vi "Frame.Settings.vi"(6 "Action":enum8{"Get", "Set"}(ring), 8 "error in (no error)":errorcluster, 10 "Frame.Settings":T1={"ID"=0, "Disable Transmission"=FALSE, "Disable Transmission Ref"=18446744073709551615, "Transmit Trigger"=enum."Channel value change", "Transmit Trigger Ref"=18446744073709551615} {"Transmit Trigger Ref" format="%.0x"; "Disable Transmission Ref" format="%.0x"}, 11 "Item Ref in":T2 format="%.0x") -> (0 "error out":errorcluster, 2 "Frame.Settings":T1={"ID"=0, "Disable Transmission"=FALSE, "Disable Transmission Ref"=18446744073709551615, "Transmit Trigger"=enum."Channel value change", "Transmit Trigger Ref"=18446744073709551615} {"Transmit Trigger Ref" format="%.0x"; "Disable Transmission Ref" format="%.0x"}, 3 "Item Ref out":T2 format="%.0x")   [LabVIEW 2025, in "Protection and Counter Addon System Explorer.lvlib"]
uses:
  Protection and Counter Addon System Explorer.lvlib
  <vilib>/NI VeriStand/Custom Device API/Custom Device Item Ref.ctl
  Types/Frame Settings.ctl
  Types/Event Trigger Type.ctl
  Addon Shared/SubVIs/GUID Lookup.vi
  Addon Shared/Protection and Counter Addon Shared.lvlib
  <vilib>/NI/NI VeriStand Advanced SysDef API/SysDef API/Advanced System Definition.lvlib
  <vilib>/NI/NI VeriStand Advanced SysDef API/_SubVIs/SysDef.Property.Get.U32.vi
  <vilib>/NI/NI VeriStand Advanced SysDef API/_SubVIs/SysDef.Property.Get.Boolean.vi
  <vilib>/NI/NI VeriStand Advanced SysDef API/_SubVIs/SysDef.Property.Set.U32.vi
  <vilib>/NI/NI VeriStand Advanced SysDef API/_SubVIs/SysDef.Property.Set.Boolean.vi
  <vilib>/NI/NI VeriStand Advanced SysDef API/_SubVIs/SysDef.Property.Set.Node.vi
  <vilib>/NI/NI VeriStand Advanced SysDef API/_SubVIs/SysDef.Search.Parent.vi
  <vilib>/NI/NI VeriStand Advanced SysDef API/_SubVIs/SysDef.Property.Get.Node.vi
  <vilib>/NI VeriStand/Custom Device API/Custom Device API.lvlib
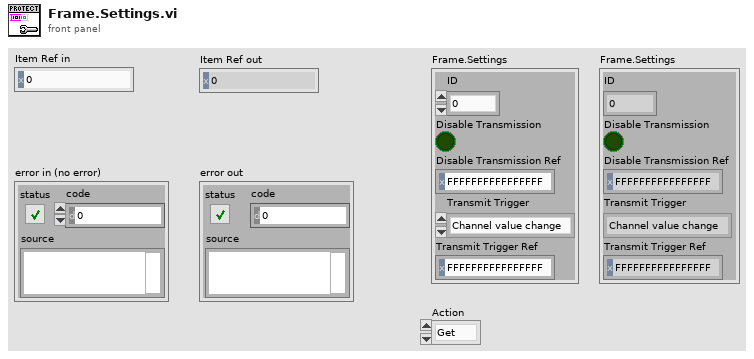
[diagram p1: front panel]
types:
  T1 = typedef "Protection and Counter Addon System Explorer.lvlib/Frame Settings.ctl" = cluster{"ID":u32, "Disable Transmission":bool, "Disable Transmission Ref":T2, "Transmit Trigger":T3, "Transmit Trigger Ref":T2}
  T2 = typedef "Custom Device API.lvlib/Custom Device Item Ref.ctl" = u64
  T3 = typedef "Protection and Counter Addon System Explorer.lvlib/Event Trigger Type.ctl" = enum16{"Channel value change", "Trigger channel (not zero)", "Channel value change or trigger channel (not zero)", "Trigger channel (any value change)", "Channel value change or trigger channel (any value change)"}
  T4 = typedef "Advanced System Definition.lvlib/TreeItem.Info.ctl" = cluster{"Name":string, "Description":string, "GUID":string, "Is Channel":bool, "Channel":T5, "Is Waveform":bool, "Waveform":T7}
  T5 = typedef "Custom Device API.lvlib/Custom Device Channel.ctl" = cluster{"Type":T6, "Units":string, "Default Value":dbl, "Faultable":bool, "Scalable":bool}
  T6 = typedef "Custom Device API.lvlib/Custom Device Channel Type.ctl" = enum16{"Input", "Output"}
  T7 = typedef "Custom Device API.lvlib/Custom Device Waveform.ctl" = cluster{"Data Type":T8, "Units":string}
  T8 = typedef "Custom Device API.lvlib/Custom Device Waveform DataType.ctl" = enum16{"Double", "Complex Double"}
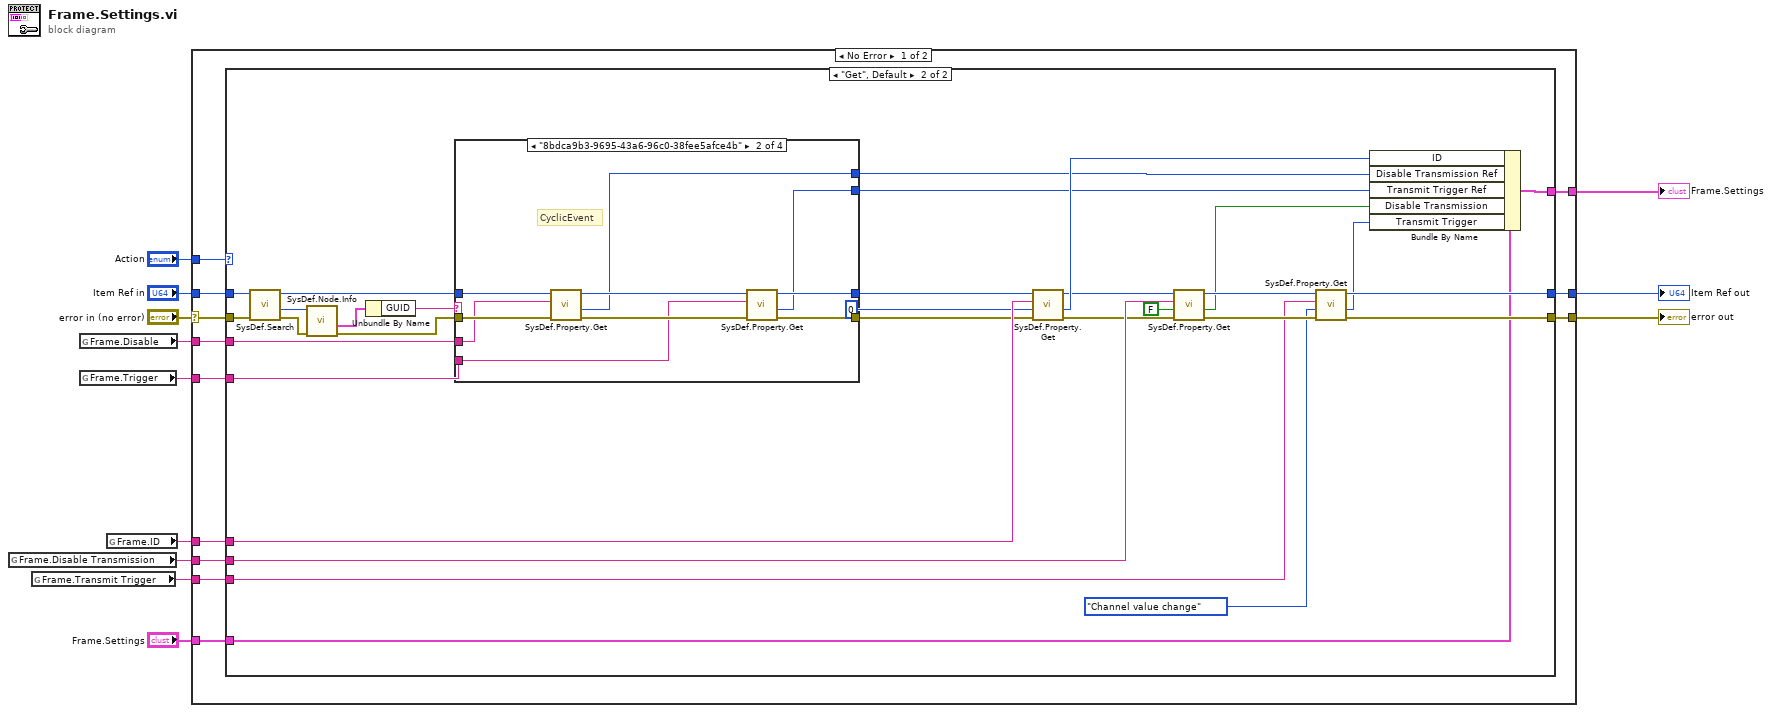
[diagram p0: block diagram]
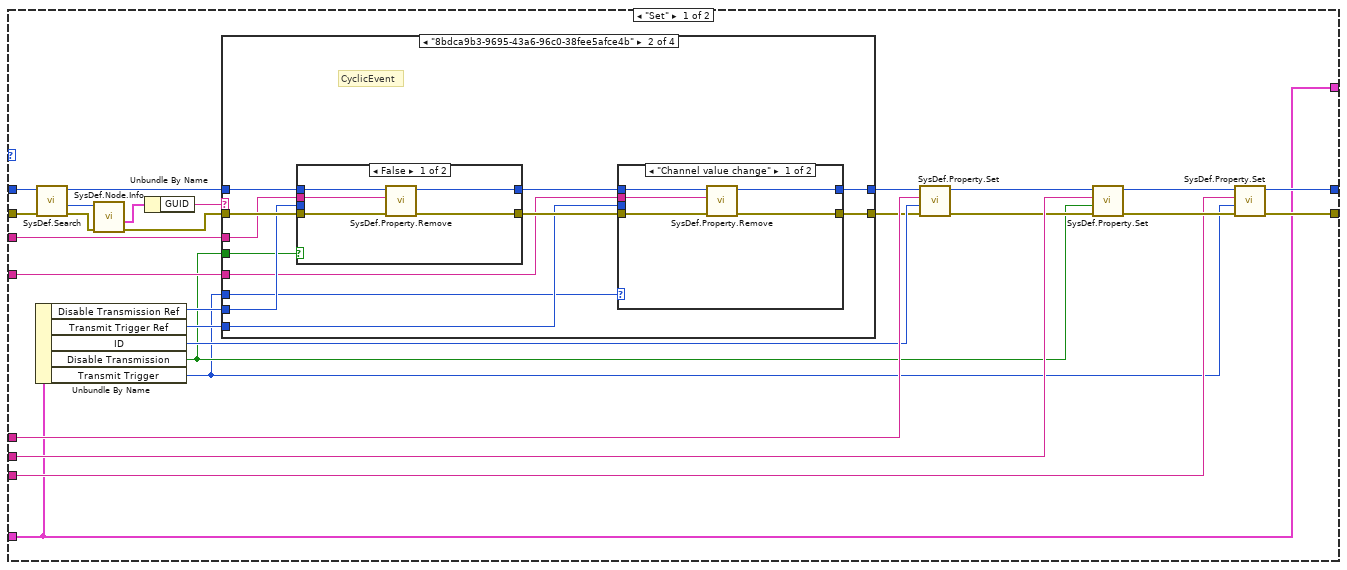
[diagram p2: hidden frame]
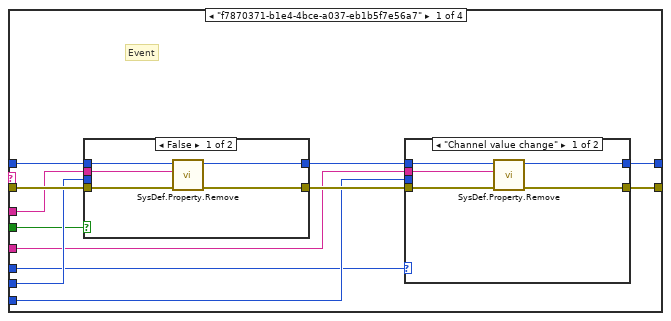
[diagram p3: hidden frame]
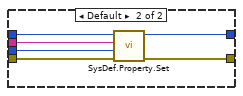
[diagram p4: hidden frame]
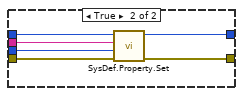
[diagram p5: hidden frame]
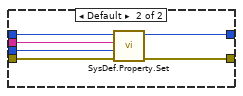
[diagram p6: hidden frame]
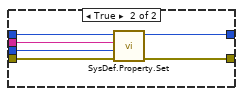
[diagram p7: hidden frame]
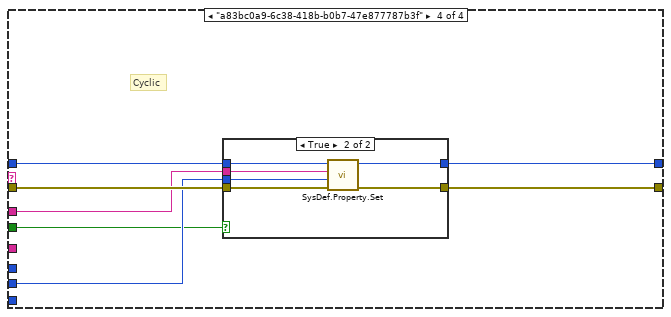
[diagram p9: hidden frame]
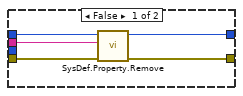
[diagram p10: hidden frame]
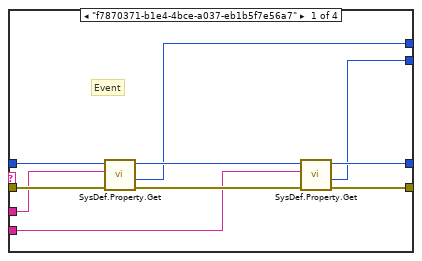
[diagram p11: hidden frame]
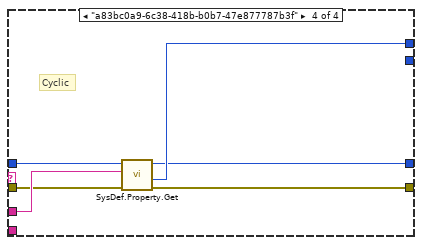
[diagram p13: hidden frame]
diagram:
  n1 = global read "GUID Lookup.vi" "Frame.Disable Transmission"() -> (w4:string)
  n2 = global read "GUID Lookup.vi" "Frame.Transmit Trigger"() -> (w5:string)
  n3 = global read "GUID Lookup.vi" "Frame.Disable"() -> (w1:string)
  n4 = global read "GUID Lookup.vi" "Frame.Trigger"() -> (w2:string)
  n5 = global read "GUID Lookup.vi" "Frame.ID"() -> (w3:string)
  n6 = case shown="No Error" "error in (no error)" {
    selector: "error in (no error)" -> [w15 w199]
    tunnel: "Item Ref in" -> [w24 w198]
    tunnel: w3 -> [w23 _]
    tunnel: w1 -> [w22 _]
    tunnel: w2 -> [w21 _]
    tunnel: [w20 w199] -> w11
    tunnel: [w19 w198] -> w10
    tunnel: [w18 _] -> w9
    tunnel: w5 -> [w17 _]
    tunnel: w4 -> [w16 _]
    tunnel: "Frame.Settings" -> [w14 _]
    tunnel: "Action" -> [w13 _]
    frame No Error {
      n7 = case shown="\"Get\", Default" w13 {
        tunnel: w24 -> [w37 w149]
        tunnel: w23 -> [w50 w169]
        tunnel: w22 -> [w34 w144]
        tunnel: w21 -> [w33 w143]
        tunnel: [w47 w165] -> w20
        tunnel: [w46 w164] -> w19
        tunnel: [w43 w157] -> w18
        tunnel: w17 -> [w45 w163]
        tunnel: w16 -> [w44 w162]
        tunnel: w15 -> [w36 w146]
        tunnel: w14 -> [w43 w158]
        frame "Set" {
          n8 = Unbundle By Name(w43) -> ("Disable Transmission Ref"=w28:T2, "Transmit Trigger Ref"=w27:T2, "ID"=w42:u32, "Disable Transmission"=w26:bool, "Transmit Trigger"=w25:T3)
          n9 = call-poly <vilib>:"SysDef.Search.vi"("error in (no error)"=w36, "nodeID"=w37) -> ("error out"=w32:errorcluster, "Value out"=w39:u64, "nodeID out"=w38:u64)  [unwired: 6 in, 1 out]
          n10 = call <vilib>:"SysDef.Node.Info.vi"("error in (no error)"=w32, "nodeID"=w39) -> ("error out"=w35:errorcluster, "Item Info"=w40:T4)  [unwired: 6 in, 2 out]
          n11 = Unbundle By Name(w40) -> ("GUID"=w41:string)
          n12 = case shown="\"8bdca9b3-9695-43a6-96c0-38fee5afce4b\"" w41 {
            tunnel: w35 -> [w62 w96 w120 w127]
            tunnel: [w52 w86 w120 w122] -> w31
            tunnel: w34 -> [w61 w95 _ w125]
            tunnel: w33 -> [w55 w89 _ _]
            tunnel: w38 -> [w60 w94 w119 w124]
            tunnel: [w53 w87 w119 w123] -> _
            tunnel: w28 -> [w59 w93 _ w126]
            tunnel: w27 -> [w56 w90 _ _]
            tunnel: w26 -> [w58 w92 _ w121]
            tunnel: w25 -> [w51 w85 _ _]
            frame "f7870371-b1e4-4bce-a037-eb1b5f7e56a7" {
              # "Event"
              n13 = case shown="False" w58 {
                tunnel: [w74 w84] -> w54
                tunnel: [w75 w83] -> w57
                tunnel: w62 -> [w76 w82]
                tunnel: w61 -> [w77 w81]
                tunnel: w60 -> [w78 w80]
                tunnel: w59 -> [_ w79]
                frame False {
                  n14 = call <vilib>:"SysDef.Property.Remove.vi"("error in (no error)"=w76, "Property Name"=w77, "nodeID"=w78) -> ("error out"=w75:errorcluster, "nodeID out"=w74:u64)  [unwired: 6 in, 1 out]
                }
                frame True {
                  n15 = call-poly <vilib>:"SysDef.Property.Set.vi"("error in (no error)"=w82, "Value"=w79, "Property Name"=w81, "nodeID"=w80) -> ("error out"=w83:errorcluster, "nodeID out"=w84:u64)  [unwired: 6 in]
                }
              }
              n16 = case shown="\"Channel value change\"" w51 {
                tunnel: [w63 w73] -> w53
                tunnel: [w64 w72] -> w52
                tunnel: w57 -> [w65 w71]
                tunnel: w55 -> [w66 w70]
                tunnel: w54 -> [w67 w69]
                tunnel: w56 -> [_ w68]
                frame "Channel value change" {
                  n17 = call <vilib>:"SysDef.Property.Remove.vi"("error in (no error)"=w65, "Property Name"=w66, "nodeID"=w67) -> ("error out"=w64:errorcluster, "nodeID out"=w63:u64)  [unwired: 6 in, 1 out]
                }
                frame Default {
                  n18 = call-poly <vilib>:"SysDef.Property.Set.vi"("error in (no error)"=w71, "Value"=w68, "Property Name"=w70, "nodeID"=w69) -> ("error out"=w72:errorcluster, "nodeID out"=w73:u64)  [unwired: 6 in]
                }
              }
            }
            frame "8bdca9b3-9695-43a6-96c0-38fee5afce4b" {
              # "CyclicEvent"
              n19 = case shown="False" w92 {
                tunnel: [w108 w118] -> w88
                tunnel: [w109 w117] -> w91
                tunnel: w96 -> [w110 w116]
                tunnel: w95 -> [w111 w115]
                tunnel: w94 -> [w112 w114]
                tunnel: w93 -> [_ w113]
                frame False {
                  n20 = call <vilib>:"SysDef.Property.Remove.vi"("error in (no error)"=w110, "Property Name"=w111, "nodeID"=w112) -> ("error out"=w109:errorcluster, "nodeID out"=w108:u64)  [unwired: 6 in, 1 out]
                }
                frame True {
                  n21 = call-poly <vilib>:"SysDef.Property.Set.vi"("error in (no error)"=w116, "Value"=w113, "Property Name"=w115, "nodeID"=w114) -> ("error out"=w117:errorcluster, "nodeID out"=w118:u64)  [unwired: 6 in]
                }
              }
              n22 = case shown="\"Channel value change\"" w85 {
                tunnel: [w97 w107] -> w87
                tunnel: [w98 w106] -> w86
                tunnel: w91 -> [w99 w105]
                tunnel: w89 -> [w100 w104]
                tunnel: w88 -> [w101 w103]
                tunnel: w90 -> [_ w102]
                frame "Channel value change" {
                  n23 = call <vilib>:"SysDef.Property.Remove.vi"("error in (no error)"=w99, "Property Name"=w100, "nodeID"=w101) -> ("error out"=w98:errorcluster, "nodeID out"=w97:u64)  [unwired: 6 in, 1 out]
                }
                frame Default {
                  n24 = call-poly <vilib>:"SysDef.Property.Set.vi"("error in (no error)"=w105, "Value"=w102, "Property Name"=w104, "nodeID"=w103) -> ("error out"=w106:errorcluster, "nodeID out"=w107:u64)  [unwired: 6 in]
                }
              }
            }
            frame "45d997b9-be87-4536-8aa7-486032a53b20", Default {
              # "SinglePoint"
            }
            frame "a83bc0a9-6c38-418b-b0b7-47e877787b3f" {
              # "Cyclic"
              n25 = case shown="True" w121 {
                tunnel: [w128 w138] -> w123
                tunnel: [w129 w137] -> w122
                tunnel: w127 -> [w130 w136]
                tunnel: w125 -> [w131 w135]
                tunnel: w124 -> [w132 w134]
                tunnel: w126 -> [_ w133]
                frame False {
                  n26 = call <vilib>:"SysDef.Property.Remove.vi"("error in (no error)"=w130, "Property Name"=w131, "nodeID"=w132) -> ("error out"=w129:errorcluster, "nodeID out"=w128:u64)  [unwired: 6 in, 1 out]
                }
                frame True {
                  n27 = call-poly <vilib>:"SysDef.Property.Set.vi"("error in (no error)"=w136, "Value"=w133, "Property Name"=w135, "nodeID"=w134) -> ("error out"=w137:errorcluster, "nodeID out"=w138:u64)  [unwired: 6 in]
                }
              }
            }
          }
          n28 = call-poly <vilib>:"SysDef.Property.Set.vi"("error in (no error)"=w31, "Value"=w42, "Property Name"=w50, "nodeID"=w37) -> ("error out"=w30:errorcluster, "nodeID out"=w29:u64)  [unwired: 6 in]
          n29 = call-poly <vilib>:"SysDef.Property.Set.vi"("error in (no error)"=w30, "Value"=w26, "Property Name"=w44, "nodeID"=w29) -> ("error out"=w48:errorcluster, "nodeID out"=w49:u64)  [unwired: 6 in]
          n30 = call-poly <vilib>:"SysDef.Property.Set.vi"("error in (no error)"=w48, "Value"=w25, "Property Name"=w45, "nodeID"=w49) -> ("error out"=w47:errorcluster, "nodeID out"=w46:u64)  [unwired: 6 in]
        }
        frame "Get", Default {
          n31 = call-poly <vilib>:"SysDef.Search.vi"("error in (no error)"=w146, "nodeID"=w149) -> ("error out"=w150:errorcluster, "Value out"=w151:u64, "nodeID out"=w142:u64)  [unwired: 6 in, 1 out]
          n32 = call <vilib>:"SysDef.Node.Info.vi"("error in (no error)"=w150, "nodeID"=w151) -> ("error out"=w152:errorcluster, "Item Info"=w153:T4)  [unwired: 6 in, 2 out]
          n33 = Unbundle By Name(w153) -> ("GUID"=w154:string)
          n34 = case shown="\"8bdca9b3-9695-43a6-96c0-38fee5afce4b\"" w154 {
            tunnel: w152 -> [w177 w187 w191 w195]
            tunnel: [w176 w186 w191 w194] -> w145
            tunnel: w144 -> [w175 w185 _ w197]
            tunnel: w143 -> [w174 w184 _ _]
            tunnel: w142 -> [w173 w183 w190 w196]
            tunnel: [w172 w182 w190 w192] -> w141
            tunnel: [w171 w181 _ w193] -> w140
            tunnel: [w170 w180 _ _] -> w139
            frame "f7870371-b1e4-4bce-a037-eb1b5f7e56a7" {
              # "Event"
              n35 = call-poly <vilib>:"SysDef.Property.Get.vi"("error in (no error)"=w177, "Property Name"=w175, "nodeID"=w173) -> ("error out"=w178:errorcluster, "Value out"=w171:u64, "nodeID out"=w179:u64)  [unwired: 5 in, 1 out]
              n36 = call-poly <vilib>:"SysDef.Property.Get.vi"("error in (no error)"=w178, "Property Name"=w174, "nodeID"=w179) -> ("error out"=w176:errorcluster, "Value out"=w170:u64, "nodeID out"=w172:u64)  [unwired: 5 in, 1 out]
            }
            frame "8bdca9b3-9695-43a6-96c0-38fee5afce4b" {
              # "CyclicEvent"
              n37 = call-poly <vilib>:"SysDef.Property.Get.vi"("error in (no error)"=w187, "Property Name"=w185, "nodeID"=w183) -> ("error out"=w188:errorcluster, "Value out"=w181:u64, "nodeID out"=w189:u64)  [unwired: 5 in, 1 out]
              n38 = call-poly <vilib>:"SysDef.Property.Get.vi"("error in (no error)"=w188, "Property Name"=w184, "nodeID"=w189) -> ("error out"=w186:errorcluster, "Value out"=w180:u64, "nodeID out"=w182:u64)  [unwired: 5 in, 1 out]
            }
            frame "45d997b9-be87-4536-8aa7-486032a53b20", Default {
              # "SinglePoint"
            }
            frame "a83bc0a9-6c38-418b-b0b7-47e877787b3f" {
              # "Cyclic"
              n39 = call-poly <vilib>:"SysDef.Property.Get.vi"("error in (no error)"=w195, "Property Name"=w197, "nodeID"=w196) -> ("error out"=w194:errorcluster, "Value out"=w193:u64, "nodeID out"=w192:u64)  [unwired: 5 in, 1 out]
            }
          }
          n40 = call-poly <vilib>:"SysDef.Property.Get.vi"("error in (no error)"=w145, "Value"=u32 0 ("Default Value"), "Property Name"=w169, "nodeID"=w141) -> ("error out"=w148:errorcluster, "Value out"=w161:u32, "nodeID out"=w147:u64)  [unwired: 4 in, 1 out]
          n41 = call-poly <vilib>:"SysDef.Property.Get.vi"("error in (no error)"=w148, "Value"=FALSE ("Default Value"), "Property Name"=w162, "nodeID"=w147) -> ("error out"=w166:errorcluster, "Value out"=w159:bool, "nodeID out"=w167:u64)  [unwired: 4 in, 1 out]
          n42 = call-poly <vilib>:"SysDef.Property.Get.vi"("error in (no error)"=w166, "Value"=Event_Trigger_Type."Channel value change" ("Transmit Trigger"), "Property Name"=w163, "nodeID"=w167) -> ("error out"=w165:errorcluster, "Value out"=w160:u32, "nodeID out"=w164:u64)  [unwired: 4 in, 1 out]
          n43 = Bundle By Name(cluster=w158, "ID"=w161, "Disable Transmission Ref"=w140, "Transmit Trigger Ref"=w139, "Disable Transmission"=w159, "Transmit Trigger"=w160) -> (w157:T1)
        }
      }
    }
    frame Error {
    }
  }
  "Item Ref out" <- w10
  "error out" <- w11
  "Frame.Settings" <- w9
